vi "query HO Uplink Channel.vi"(8 "error in (no error)":errorcluster caption="에러 입력(에러 없음)", 9 "UL Channel Arguments":T2, 11 "LTE 입력":refnum<class "LTE.lvclass">) -> (0 "error out":errorcluster caption="에러 출력", 2 "UL Channel Info":T1, 3 "LTE 출력":refnum<class "LTE.lvclass">)   [LabVIEW 2023, in "ANRITSU Call Box.lvlib" / "LTE.lvclass"]
uses:
  LTE.lvclass
  LTE.lvclass/LTE.ctl
  ANRITSU Call Box.lvlib
  Type Definition/LTE Uplink Channel Number Info.ctl
  Type Definition/LTE Uplink Channel Number Target.ctl
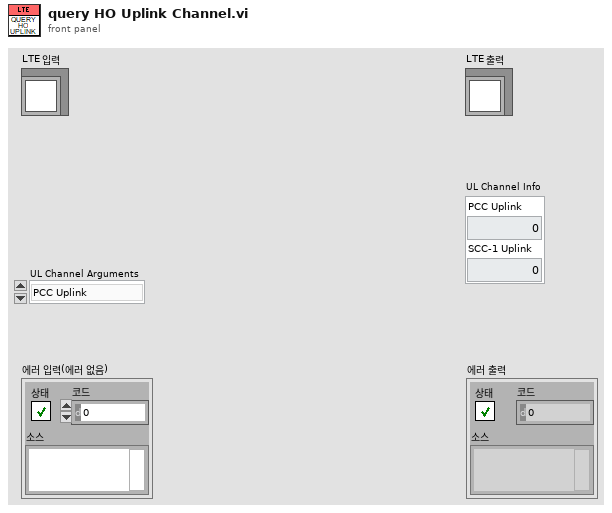
[diagram p1: front panel]
types:
  T1 = typedef "ANRITSU Call Box.lvlib/LTE Uplink Channel Number Info.ctl" = cluster{"PCC Uplink":i32, "SCC-1 Uplink":i32}
  T2 = typedef "ANRITSU Call Box.lvlib/LTE Uplink Channel Number Target.ctl" = enum16{"PCC Uplink", "SCC-1 Uplink", "All"}
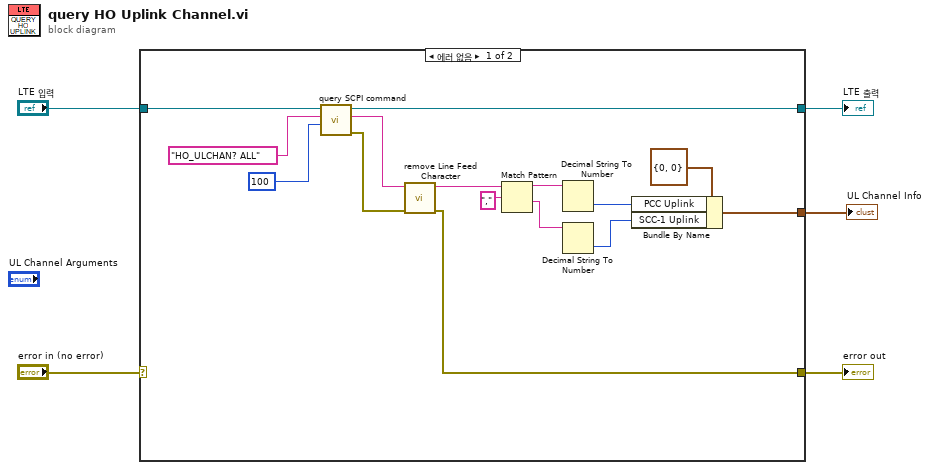
[diagram p0: block diagram]
diagram:
  n1 = case shown="에러 없음" "error in (no error)" {
    selector: "error in (no error)" -> [_ w22]
    tunnel: [w6 w22] -> w4
    tunnel: [w8 w21] -> w2
    tunnel: "LTE 입력" -> [w9 w21]
    tunnel: [w7 _] -> w1
    frame No Error {
      n2 = call "query SCPI command.vi"("Read Buffer Length"=u32 100, "SCPI Command"="HO_ULCHAN? ALL" ("string"), "LTE in"=w9) -> ("error out"=w17:errorcluster, "Read Buffer String"=w18:string, "LTE out"=w8:refnum<class "LTE.lvclass">)  [unwired: 6 in]
      n3 = call "remove Line Feed Character.vi"("error in"=w17, "Query String"=w18) -> ("error out"=w6:errorcluster, "Line Feed Removed String"=w13:string)  [unwired: 8 in]
      n4 = Match Pattern(string=w13, regular expression=",") -> (before substring=w15:string, after substring=w14:string)  [unwired: 1 in, 2 out]
      n5 = Decimal String To Number(string=w15) -> (number=w11:i32)  [unwired: 2 in, 1 out]
      n6 = Decimal String To Number(string=w14) -> (number=w10:i32)  [unwired: 2 in, 1 out]
      n7 = Bundle By Name(cluster=T1 {"PCC Uplink"=0, "SCC-1 Uplink"=0} ("UL Channel Info 2"), "PCC Uplink"=w11, "SCC-1 Uplink"=w10) -> (w7:T1)
    }
    frame Error {
    }
  }
  "error out" <- w4
  "LTE 출력" <- w2
  "UL Channel Info" <- w1
